vi "ADT RCD Current.vi"(8 "error in":errorcluster) -> (0 "error out":errorcluster, 2 "Result":string, 3 "RESULT":bool)   [LabVIEW 2021]
uses:
  DUT/DUT_Cmd.ctl
panel:
  out "number":dbl
  out "Command Response":string
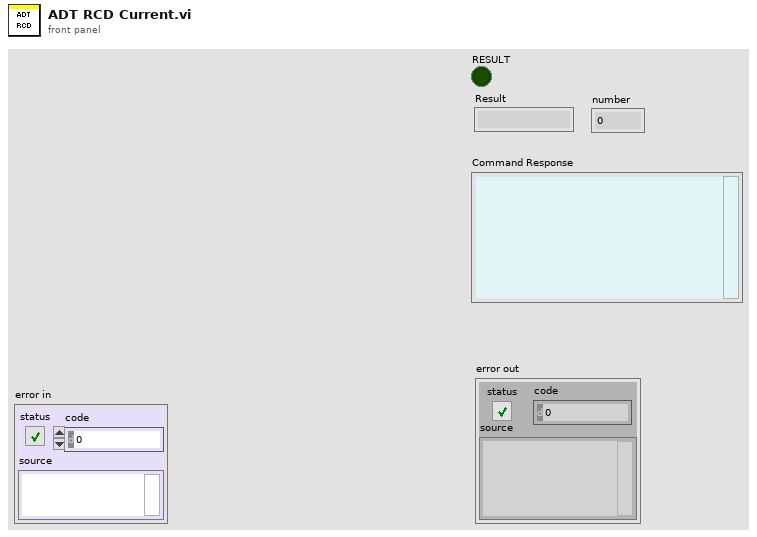
[diagram p1: front panel]
types:
  T1 = typedef "DUT_Cmd.ctl" = enum16{"Unlock serial", "Stop console logs", "Release emergency at start", "Read firmware", "WiFi credentials", "WiFi connected", "WiFi SSID", "Board revision", "ADC_NTC_TEMP", "ADC_TYPE2_RCD_CURRENT", "PCBA serial write", "PCBA serial readback", "Start energy meter", "Energy meter Vac", "Energy meter Iac", "Energy meter PF", "Energy meter energy", "Provision", "Set gateway identity", "CP checklist", "Earth detect", "D+M sense unplugged", "D+M sense plugged", "Output relay weld", "Start diagnostics", "Relay 1 on", "Relay 2 on", "Emergency pressed", "Release emergency", "Emergency released", "Unlock serial for 5 A", "Board current (5 A)", "Unlock serial for 15 A", "Board current (15 A)", "Unlock serial for 0 A", "NFC tag", "Start diagnostics again", "Relay 2 off", "Relay 1 off", "End diagnostics", "Load current (5 A) [No USB station]", "Load current (15 A) [No USB station]", "Load current (0 A) [No USB station]", "NFC tag [No USB station]", "Battery Voltage", "FW Power reset", "Notification LED", "O/P Relay weld Detection", "Earth Detection", "12V ", "5V", "3.3V"}
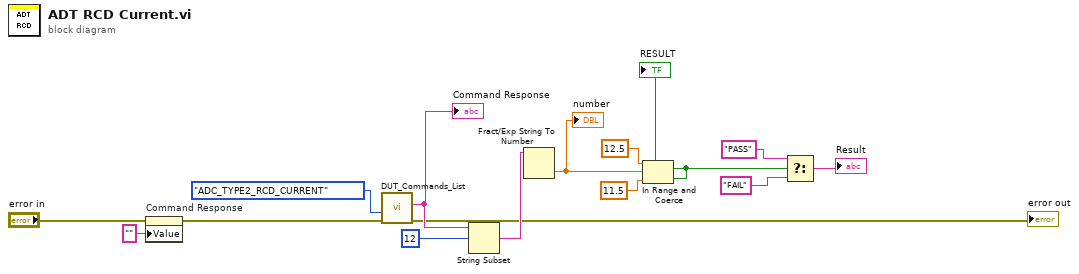
[diagram p0: block diagram]
diagram:
  n1 = property on="Command Response" class="Str"(error in="error in", "Value"="" ("Command Response")) -> (error out=w10:errorcluster)  [unwired: 1 in, 1 out]
  n2 = call "DUT_Commands_List.vi"("error in"=w10, "DUT Cmd"=DUT_Cmd."ADC_TYPE2_RCD_CURRENT") -> ("error out"=→"error out":errorcluster, "Command Response"=w4:string)  [unwired: 7 in, 1 out]
  "Command Response" <- w4
  n3 = String Subset(string=w4, offset (0)=12) -> (substring=w2:string)  [unwired: 1 in]
  n4 = Fract/Exp String To Number(string=w2) -> (number=w8:dbl)  [unwired: 3 in, 1 out]
  "number" <- w8
  n5 = In Range and Coerce(upper limit=12.5, x=w8, lower limit=11.5) -> (In Range?=w5:bool)  [unwired: 1 out]
  "RESULT" <- w5
  n6 = Select(t="PASS", s=w5, f="FAIL") -> (s? t:f=→"Result":string)
